vi "Create ConfigDataDVR.vi"(8 "error in (no error)":errorcluster, 11 "Settings":T1) -> (0 "error out":errorcluster)   [LabVIEW 2019, in "Language Selection.lvlib"]
doc: "Converts the translation data into a Data Value Reference.\n- - -\nCopyright (c) 2026, Merecs Engineering GmbH"
uses:
  Language Selection.lvlib
  TypeDefs/Cluster Language Configuration.ctl
  community/Cluster Settings Data.ctl
  TypeDefs/Cluster Language.ctl
  TypeDefs/Cluster PropertyTranslation.ctl
  TypeDefs/Enum Property Type.ctl
  Cluster DVR.ctl
  TypeDefs/Cluster LanguageClusterWithRefnum.ctl
  Global Language Selection.vi
panel:
  # "Connector Pane"
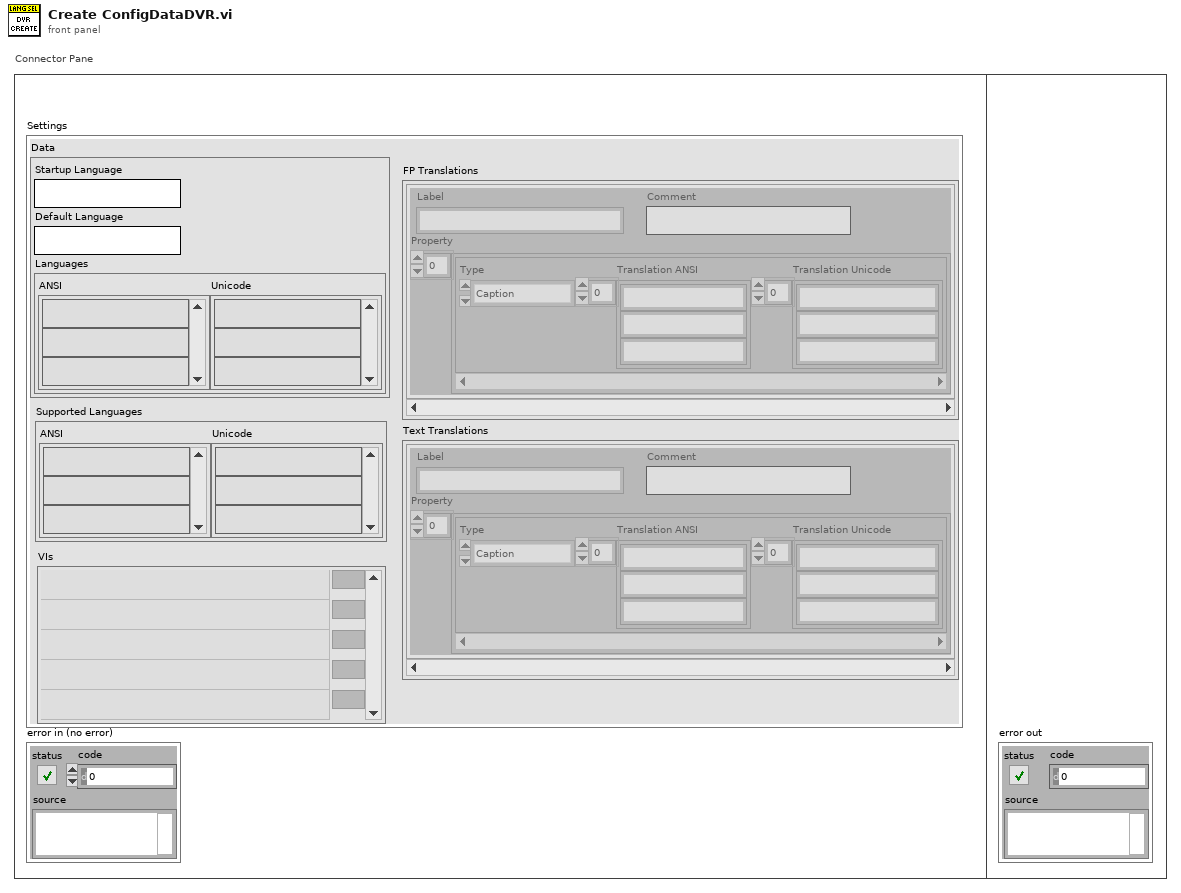
[diagram p1: front panel]
types:
  T1 = typedef "Language Selection.lvlib/Cluster Language Configuration.ctl" = cluster{"Data":T2, "Supported Languages":cluster{"ANSI":string[], "Unicode":string[]}, "VIs":path[], "FP Translations":T3[], "Text Translations":T3[]}
  T2 = typedef "Language Selection.lvlib/Cluster Settings Data.ctl" = cluster{"Startup Language":string, "Default Language":string, "Languages":cluster{"ANSI":string[], "Unicode":string[]}}
  T3 = typedef "Language Selection.lvlib/Cluster Language.ctl" = cluster{"Label":string, "Comment":string, "Property":T4[]}
  T4 = typedef "Language Selection.lvlib/Cluster PropertyTranslation.ctl" = cluster{"Type":T5, "Translation ANSI":string[], "Translation Unicode":string[]}
  T5 = typedef "Language Selection.lvlib/Enum Property Type.ctl" = enum16{"NA", "Caption", "String Value", "Boolean Text", "Ring Strings", "1D Array Elements", "2D Array Elements", "(MC)Listbox Header", "(MC)Listbox Items", "Tab Pages Names", "X & Y GraphChart", "Plot Names", "Table Headers", "Table Items", "TipStrip", "Combobox Strings", "Cursor Name", "Tree Col Headers"}
  T6 = typedef "Language Selection.lvlib/Cluster LanguageClusterWithRefnum.ctl" = cluster{"Property":T4[], "Controls":set{refnum<vi>}}
  T7 = typedef "Language Selection.lvlib/Cluster DVR.ctl" = cluster{"Data":T2, "VIs":path[], "FP Translation":map{string, T6}, "Text Translation":map{string, T6}, "Front panels":set{refnum<vi>}}
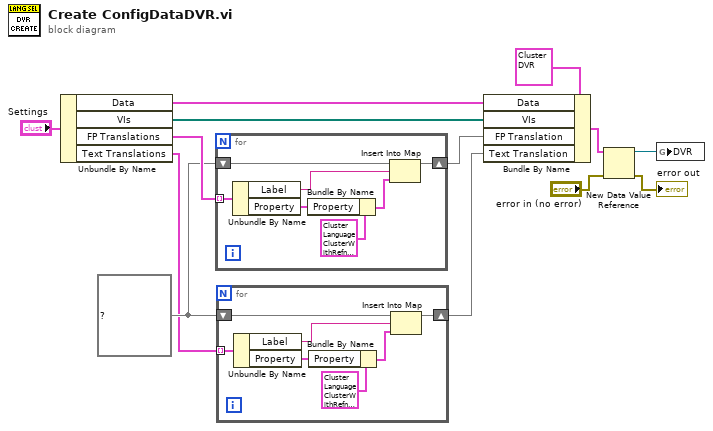
[diagram p0: block diagram]
diagram:
  w3 = map{string, T6} {} ("CTRL Translation")
  n1 = Unbundle By Name("Settings") -> ("Data"=w6:T2, "VIs"=w5:path[], "FP Translations"=w13:T3[], "Text Translations"=w1:T3[])
  n2 = for {
    tunnel: w13 -> [w20] mode=indexing
    shift-right: [w17] -> w4
    shift-left: w3 -> [w19]
    n3 = Unbundle By Name(w20) -> ("Label"=w18:string, "Property"=w15:T4[])
    n4 = Bundle By Name(cluster=T6 {"Property"=[], "Controls"={}} ("Translation"), "Property"=w15) -> (w14:T6)
    n5 = Insert Into Map(map in=w19, key=w18, value=w14) -> (map out=w17:map{string, T6})  [unwired: 2 out]
  }
  n6 = for {
    tunnel: w1 -> [w27] mode=indexing
    shift-right: [w24] -> w2
    shift-left: w3 -> [w26]
    n7 = Unbundle By Name(w27) -> ("Label"=w25:string, "Property"=w22:T4[])
    n8 = Bundle By Name(cluster=T6 {"Property"=[], "Controls"={}} ("Translation"), "Property"=w22) -> (w21:T6)
    n9 = Insert Into Map(map in=w26, key=w25, value=w21) -> (map out=w24:map{string, T6})  [unwired: 2 out]
  }
  n10 = Bundle By Name(cluster=T7 {"Data"={"Startup Language"="", "Default Language"="", "Languages"={"ANSI"=[], "Unicode"=[]}}, "VIs"=[], "FP Translation"={}, "Text Translation"={}, "Front panels"={}}, "Data"=w6, "VIs"=w5, "FP Translation"=w4, "Text Translation"=w2) -> (w10:T7)
  n11 = New Data Value Reference(data value=w10, error in="error in (no error)") -> (data value reference=w8:refnum<data-value>, error out=→"error out":errorcluster)
  n12 = global write "Global Language Selection.vi" "DVR"(w8) -> ()
